vi "Send I2C Transaction.vi"(8 "Error In":errorcluster, 10 "I2C Command":T1 {"Slave Address" format="%.0x"; "Register Address" format="%.0x"; "Data" format="%.0x"}, 11 "FPGA Ref in":refnum<k20>) -> (0 "Error Out":errorcluster, 2 "Read Data":u8 format="%.0x", 3 "FPGA Ref out":refnum<k20>)   [LabVIEW 2025, in "I2C Bus Monitor.lvclass"]
uses:
  I2C Bus Monitor.lvclass
  <instrlib>/FlexRIO/API/Host/v1/NI FlexRIO API v1.lvlib
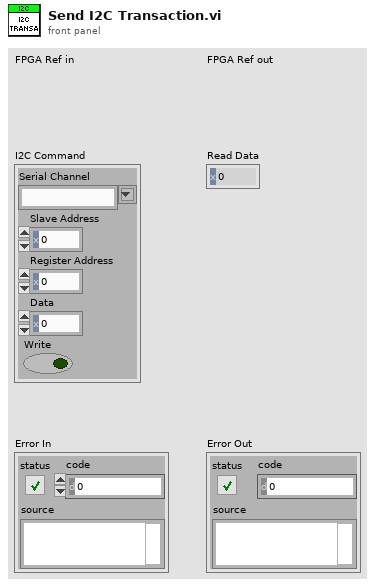
[diagram p1: front panel]
types:
  T1 = cluster{"Serial Channel":string, "Slave Address":u8, "Register Address":u16, "Data":u8, "Write":bool}
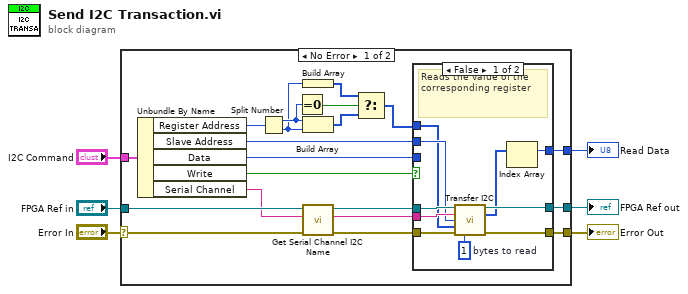
[diagram p0: block diagram]
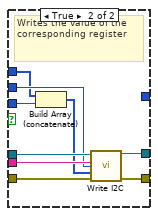
[diagram p2: hidden frame]
diagram:
  n1 = case shown="No Error" "Error In" {
    selector: "Error In" -> [w23 w46]
    tunnel: "FPGA Ref in" -> [w26 w47]
    tunnel: [w25 w47] -> w2
    tunnel: "I2C Command" -> [w13 _]
    tunnel: [w24 w46] -> w5
    tunnel: [w22 _] -> w1
    frame No Error {
      n2 = Unbundle By Name(w13) -> ("Register Address"=w21:u16, "Slave Address"=w11:u8, "Data"=w20:u8, "Write"=w12:bool, "Serial Channel"=w7:string)
      n3 = Split Number(x=w21) -> (hi(x)=w16:u8, lo(x)=w14:u8)
      n4 = Equal To 0?(x=w16) -> (x = 0?=w17:bool)
      n5 = Build Array(w14) -> (w18:u8[])
      n6 = Build Array(w16, w14) -> (w19:u8[])
      n7 = call "Get Serial Channel I2C Name.vi"("error in (no error)"=w23, "Serial Channel"=w7, "FGPA Ref in"=w26) -> ("error out"=w10:errorcluster, "SO/SI I2C Name"=w8:string, "FPGA Ref out"=w9:refnum<k20>)  [unwired: 6 in]
      n8 = Select(t=w18, s=w17, f=w19) -> (s? t:f=w15:u8[])
      n9 = case shown="False" w12 {
        tunnel: [w33 w41] -> w25
        tunnel: [w32 w40] -> w24
        tunnel: w9 -> [w36 w45]
        tunnel: w10 -> [w35 w44]
        tunnel: w8 -> [w34 w43]
        tunnel: w11 -> [w31 w38]
        tunnel: w20 -> [_ w39]
        tunnel: w15 -> [w30 w37]
        tunnel: [w28 _] -> w22
        frame False {
          w27 = u32 1  # bytes to read
          # "Reads the value of the corresponding register"
          n10 = call <instrlib>:"Transfer I2C.vi"("fpga interface in"=w36, "bus instance name"=w34, "slave address"=w31, "write data"=w30, "error in"=w35, "num bytes to read"=w27) -> ("fpga interface out"=w33:refnum<k20>, "read data"=w29:u8[], "error out"=w32:errorcluster)  [unwired: 6 in, 1 out]
          n11 = Index Array(array=w29) -> (element=w28:u8)  [unwired: 1 in]
        }
        frame True {
          # "Writes the value of the corresponding register"
          n12 = Build Array (concatenate)(w37, w39) -> (w42:u8[])
          n13 = call <instrlib>:"Write I2C.vi"("fpga interface in"=w45, "bus instance name"=w43, "slave address"=w38, "data"=w42, "error in"=w44) -> ("fpga interface out"=w41:refnum<k20>, "error out"=w40:errorcluster)  [unwired: 8 in, 1 out]
        }
      }
    }
    frame Error {
    }
  }
  "Error Out" <- w5
  "FPGA Ref out" <- w2
  "Read Data" <- w1
